vi "ValueSignalLatchBooleanArray.vi"(0 "VI Reference In":refnum<vi>, 5 "Control Path":string[](array[string]), 11 "error in":errorcluster) -> (4 "VI Reference Out":refnum<vi>, 15 "error out":errorcluster)   [LabVIEW 2016, in "Drona.lvlib" / "ControlValue.lvlib"]
doc: "Triggers the latch boolean by keyboard simulation.\n\nThe path of the control should be given in the successive index of the array"
uses:
  ControlValue.lvlib
  KeyBoardSimulation/typedef/VirtualKey.ctl
  KeyBoardSimulation/typedef/Action.ctl
  VI/MakeVIFrontMost.vi
  KeyBoardSimulation/KeyboardSimulationCore.vi
  Get/GetControlRef/GetControlRef.lvlib
  Drona.lvlib
  VI/VI.lvlib
  KeyBoardSimulation/KeyboardSimulation.lvlib
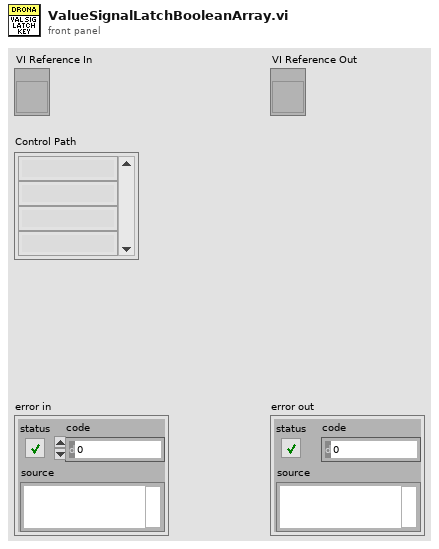
[diagram p1: front panel]
types:
  T1 = typedef "Drona.lvlib/KeyboardSimulation.lvlib/VirtualKey.ctl" = u8
  T2 = typedef "Drona.lvlib/KeyboardSimulation.lvlib/Action.ctl" = enum16{"Press", "Up", "Down"}
  T3 = cluster{"Key":T1, "Action":T2, "Delay (ms)":u32}[]
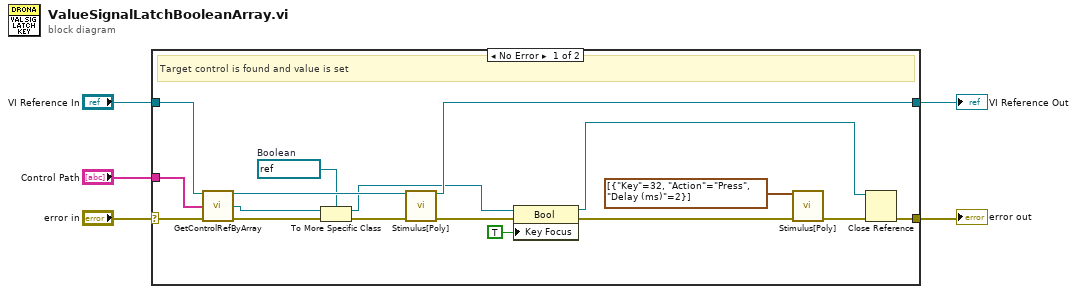
[diagram p0: block diagram]
diagram:
  n1 = case shown="No Error" "error in" {
    selector: "error in" -> [w22 w24]
    tunnel: "Control Path" -> [w20 _]
    tunnel: "VI Reference In" -> [w19 w23]
    tunnel: [w14 w23] -> w2
    tunnel: [w18 w24] -> w1
    frame No Error {
      w12 = refnum<vi> refnum  # Boolean
      # "Target control is found and value is set"
      n2 = call "GetControlRefByArray.vi"("VI Reference In"=w19, "Control Path"=w20, "error In"=w22) -> ("VI Reference Out"=w15:refnum<vi>, "Ctl Refnum"=w16:refnum<vi>, "error out"=w21:errorcluster)  [unwired: 10 in]
      n3 = To More Specific Class(target class=w12, reference=w16, error in=w21) -> (specific class reference=w11:refnum<vi>, error out=w13:errorcluster)
      n4 = call-poly "Stimulus[Poly].vi"("VI Reference In"=w15, "error in"=w13) -> ("VI Reference Out"=w14:refnum<vi>, "error out"=w10:errorcluster)  [unwired: 12 in]
      n5 = property class="Bool"(reference=w11, error in=w10, "Key Focus"=TRUE) -> (reference out=w17:refnum<vi>, error out=w6:errorcluster)
      n6 = call-poly "Stimulus[Poly].vi"("Key Array"=T3 [{"Key"=32, "Action"=enum."Press", "Delay (ms)"=2}], "error in"=w6) -> ("error out"=w7:errorcluster)  [unwired: 13 in]
      n7 = Close Reference(reference=w17, error in (no error)=w7) -> (error out=w18:errorcluster)
    }
    frame Error {
    }
  }
  "error out" <- w1
  "VI Reference Out" <- w2
